vi "AutoInstaller.vi"() -> ()   [LabVIEW 2020]
uses:
  <vilib>/zip/NI_Unzip.lvlib
panel:
  out "Text":string
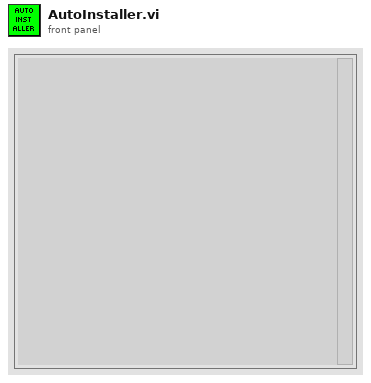
[diagram p1: front panel]
types:
  T1 = cluster{"BuildFolder":path, "Files":cluster{"ZipFile":path, "UnzippedFolder":path, "LVPath":path, "LvVer":i32, "Bit":i32}[], "LogFile":path, "pattern":string}
  T2 = cluster{"ZipFile":path, "UnzippedFolder":path, "LVPath":path, "LvVer":i32, "Bit":i32}
  T3 = cluster{"ZipFile":path, "UnzippedFolder":path, "LVPath":path, "LvVer":i32, "Bit":i32}[]
  T4 = enum32{"invalid app kind", "Development System", "Run Time System", "Student Edition", "Embedded LabVIEW", "Evaluation", "Custom"}
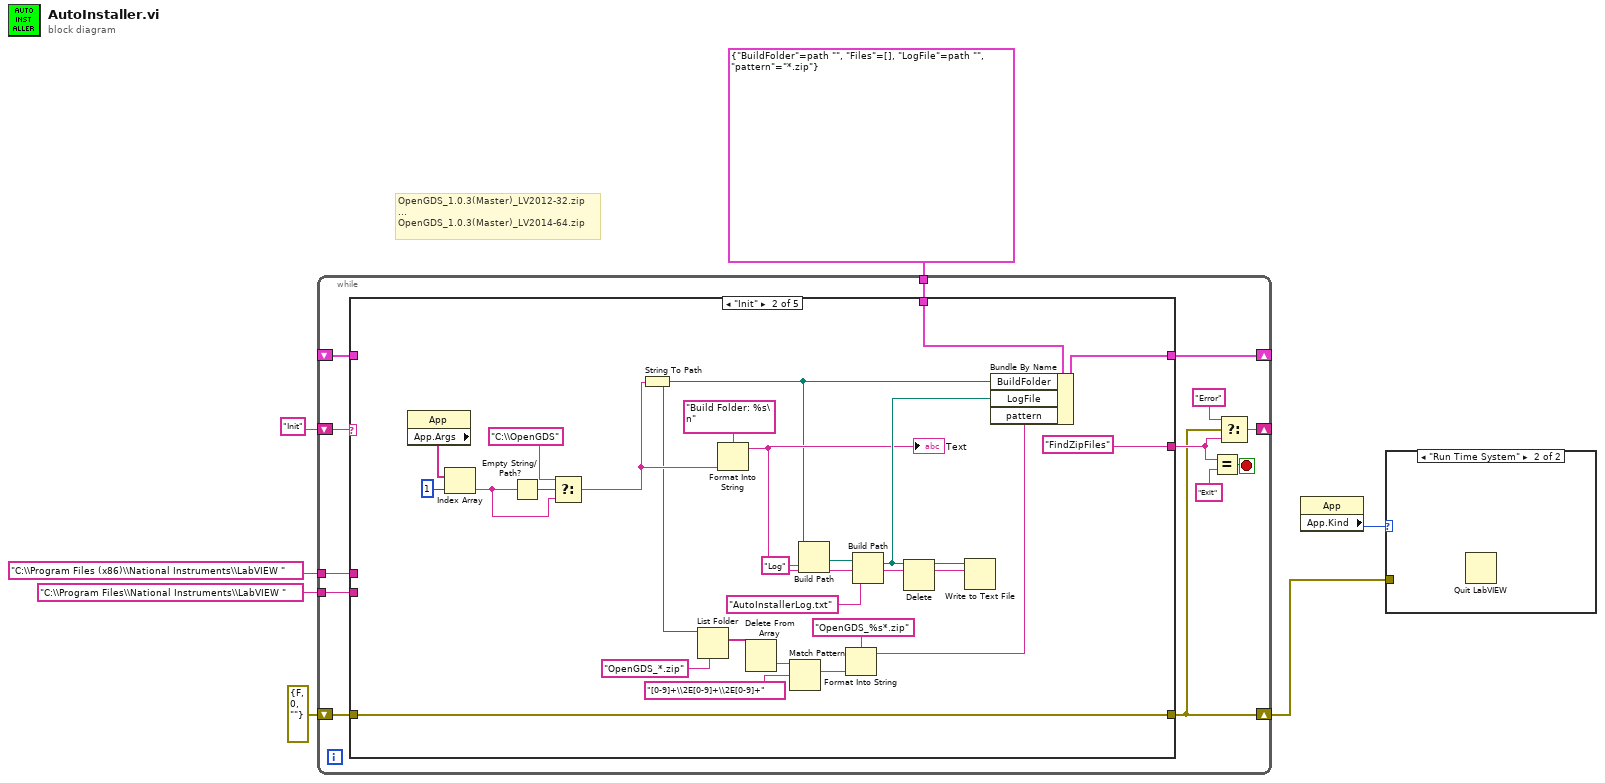
[diagram p0: block diagram]
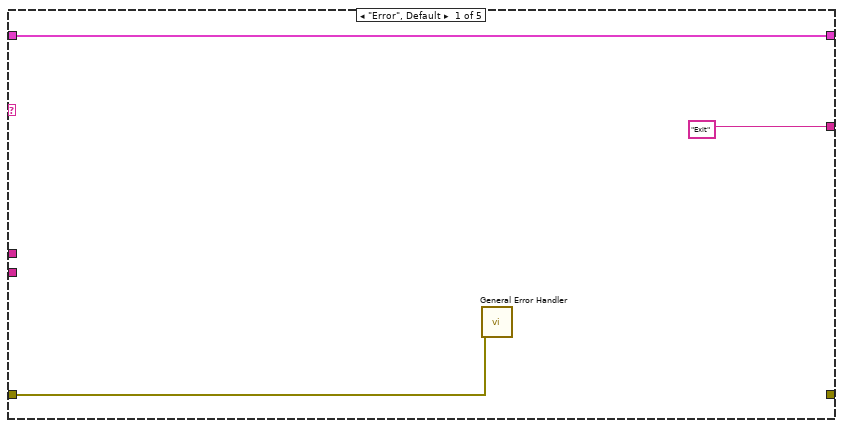
[diagram p3: hidden frame]
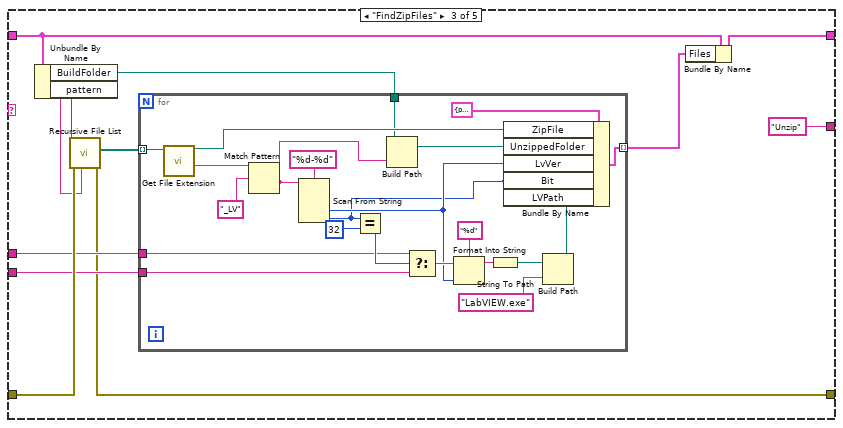
[diagram p4: hidden frame]
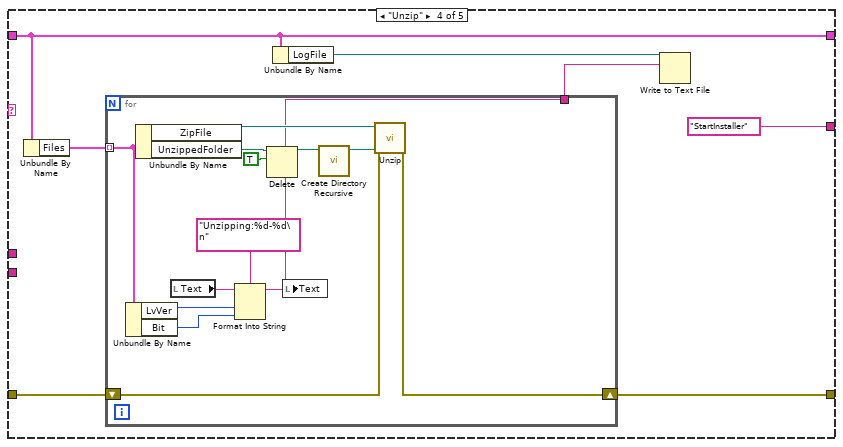
[diagram p5: hidden frame]
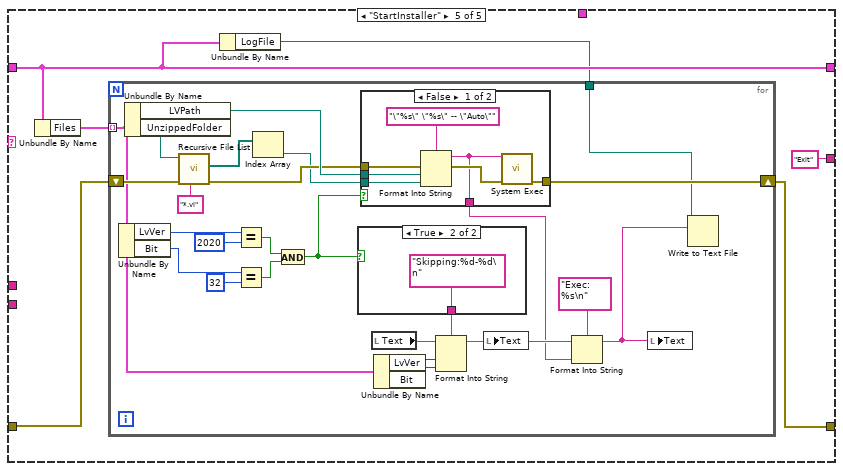
[diagram p6: hidden frame]
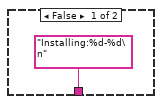
[diagram p7: hidden frame]
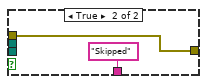
[diagram p8: hidden frame]
diagram:
  # "OpenGDS_1.0.3(Master)_LV2012-32.zip\n...\nOpenGDS_1.0.3(Master)_LV2014-64.zip"
  n1 = while {
    shift-right: [w13] -> w1
    shift-left: errorcluster {"status"=FALSE, "code"=0, "source"=""} ("error IO") -> [w20]
    shift-right: [w18] -> _
    shift-left: "Init" -> [w19]
    shift-right: [w12] -> _
    shift-left: _ -> [w11]
    tunnel: T1 {"BuildFolder"=path "", "Files"=[], "LogFile"=path "", "pattern"="*.zip"} -> [w10]
    tunnel: "C:\\Program Files (x86)\\National Instruments\\LabVIEW " -> [w9]
    tunnel: "C:\\Program Files\\National Instruments\\LabVIEW " -> [w8]
    stop <- w17 stop-if-true
    n2 = case shown="\"Init\"" w19 {
      tunnel: w20 -> [w21 w47 w56 w86 w106]
      tunnel: [_ w47 w51 w85 w104] -> w13
      tunnel: ["Exit" "FindZipFiles" "Unzip" "StartInstaller" "Exit"] -> w14
      tunnel: [w22 w46 w57 w84 w103] -> w12
      tunnel: w11 -> [w22 _ w58 w84 w103]
      tunnel: w10 -> [_ w42 _ _ _]
      tunnel: w9 -> [_ _ w54 _ _]
      tunnel: w8 -> [_ _ w53 _ _]
      frame "Error", Default {
        n3 = call <vilib>:"General Error Handler.vi"("error in (no error)"=w21) -> ()  [unwired: 10 in, 5 out]
      }
      frame "Init" {
        n4 = property class="App"() -> ("App.Args"=w43:string[])  [unwired: 2 in, 2 out]
        n5 = Index Array(array=w43, index=1) -> (element=w40:string)
        n6 = Empty String/Path?(string/path=w40) -> (empty?=w41:bool)
        n7 = Select(t="C:\\OpenGDS", s=w41, f=w40) -> (s? t:f=w39:string)
        n8 = String To Path(string=w39) -> (path=w31:path)
        n9 = List Folder(path=w31, pattern="OpenGDS_*.zip") -> (filenames=w24:string[])  [unwired: 2 in, 3 out]
        n10 = Format Into String(format string="Build Folder: %s\n", w39) -> (resulting string=w32:string)  [unwired: 2 in, 1 out]
        "Text" <- w32
        n11 = Delete From Array(array=w24) -> (deleted portion=w29:string)  [unwired: 2 in, 1 out]
        n12 = Match Pattern(string=w29, regular expression="[0-9]+\\2E[0-9]+\\2E[0-9]+") -> (match substring=w27:string)  [unwired: 1 in, 3 out]
        n13 = Build Path(base path=w31, name or relative path="Log") -> (appended path=w36:path)
        n14 = Format Into String(format string="OpenGDS_%s*.zip" ("name or relative path"), w27) -> (resulting string=w25:string)  [unwired: 2 in, 1 out]
        n15 = Build Path(base path=w36, name or relative path="AutoInstallerLog.txt") -> (appended path=w33:path)
        n16 = Delete(path (use dialog)=w33) -> (deleted path=w34:path)  [unwired: 4 in, 2 out]
        n17 = Write to Text File(file (use dialog)=w34, text=w32) -> ()  [unwired: 2 in, 3 out]
        n18 = Bundle By Name(cluster=w42, "BuildFolder"=w31, "LogFile"=w33, "pattern"=w25) -> (w46:T1)
      }
      frame "FindZipFiles" {
        n19 = Unbundle By Name(w58) -> ("BuildFolder"=w50:path, "pattern"=w49:string)
        n20 = call <vilib>:"Recursive File List.vi"("pattern"=w49, "error in (no error)"=w56, "Folder Path"=w50) -> ("error out"=w51:errorcluster, "All Files in Dir"=w55:path[])  [unwired: 4 in, 3 out]
        n21 = for {
          tunnel: w55 -> [w81] mode=indexing
          tunnel: w54 -> [w76]
          tunnel: w53 -> [w75]
          tunnel: [w65] -> w52 mode=indexing
          tunnel: w50 -> [w64]
          n22 = call <vilib>:"Get File Extension.vi"("file"=w81) -> ("filename without extension"=w60:string, "dup file"=w69:path)  [unwired: 6 in, 3 out]
          n23 = Match Pattern(string=w60, regular expression="_LV") -> (after substring=w68:string)  [unwired: 1 in, 3 out]
          n24 = Scan From String(format string="%d-%d", input string=w68) -> (output 1=w62:i32, output 2=w61:i32)  [unwired: 4 in, 3 out]
          n25 = Equal?(x=w61, y=32) -> (x = y?=w77:bool)
          n26 = Build Path(base path=w64, name or relative path=w68) -> (appended path=w67:path)
          n27 = Select(t=w76, s=w77, f=w75) -> (s? t:f=w74:string)
          n28 = Format Into String(format string="%d", initial string=w74, w62) -> (resulting string=w72:string)  [unwired: 1 in, 1 out]
          n29 = String To Path(string=w72) -> (path=w71:path)
          n30 = Build Path(base path=w71, name or relative path="LabVIEW.exe") -> (appended path=w66:path)
          n31 = Bundle By Name(cluster=T2 {"ZipFile"=path "", "UnzippedFolder"=path "", "LVPath"=path "", "LvVer"=0, "Bit"=0}, "ZipFile"=w69, "UnzippedFolder"=w67, "LvVer"=w62, "Bit"=w61, "LVPath"=w66) -> (w65:T2)
        }
        n32 = Bundle By Name(cluster=w58, "Files"=w52) -> (w57:T1)
      }
      frame "Unzip" {
        n33 = Unbundle By Name(w84) -> ("Files"=w87:T3)
        n34 = for {
          tunnel: w87 -> [w92] mode=indexing
          shift-right: [w99] -> w85
          shift-left: w86 -> [w100]
          tunnel: [w89] -> w82
          n35 = Unbundle By Name(w92) -> ("LvVer"=w91:i32, "Bit"=w90:i32)
          n36 = Unbundle By Name(w92) -> ("ZipFile"=w101:path, "UnzippedFolder"=w98:path)
          n37 = local read "Text"() -> (w94:string)
          n38 = Format Into String(format string="Unzipping:%d-%d\n", initial string=w94, w91, w90) -> (resulting string=w89:string)  [unwired: 1 in, 1 out]
          n39 = Delete(path (use dialog)=w98, entire hierarchy (F)=TRUE) -> (deleted path=w96:path)  [unwired: 3 in, 2 out]
          n40 = local write "Text"(w89) -> ()
          n41 = call <vilib>:"Create Directory Recursive.vi"("directory"=w96) -> ("directory copy"=w95:path)  [unwired: 4 in, 2 out]
          n42 = call <vilib>:"Unzip.vi"("error in (no error)"=w100, "Target directory (same as Zip file if empty)"=w95, "Zip file"=w101) -> ("error out"=w99:errorcluster)  [unwired: 6 in, 2 out]
        }
        n43 = Unbundle By Name(w84) -> ("LogFile"=w83:path)
        n44 = Write to Text File(file (use dialog)=w83, text=w82) -> ()  [unwired: 2 in, 3 out]
      }
      frame "StartInstaller" {
        n45 = Unbundle By Name(w103) -> ("Files"=w107:T3)
        n46 = Unbundle By Name(w103) -> ("LogFile"=w102:path)
        n47 = for {
          tunnel: w107 -> [w118] mode=indexing
          shift-right: [w129] -> w104
          shift-left: w106 -> [w131]
          tunnel: w102 -> [w117]
          n48 = Unbundle By Name(w118) -> ("LvVer"=w124:i32, "Bit"=w121:i32)
          n49 = Unbundle By Name(w118) -> ("LVPath"=w127:path, "UnzippedFolder"=w132:path)
          n50 = call <vilib>:"Recursive File List.vi"("pattern"="*.vi", "error in (no error)"=w131, "Folder Path"=w132) -> ("error out"=w126:errorcluster, "All Files in Dir"=w128:path[])  [unwired: 4 in, 3 out]
          n51 = Equal?(x=w124, y=2020) -> (x = y?=w120:bool)
          n52 = Equal?(x=w121, y=32) -> (x = y?=w119:bool)
          n53 = Index Array(array=w128) -> (element=w125:path)  [unwired: 1 in]
          n54 = And(x=w120, y=w119) -> (x .and. y?=w112:bool)
          n55 = case shown="True" w112 {
            tunnel: ["Installing:%d-%d\n" ("format string") "Skipping:%d-%d\n" ("format string")] -> w115
            frame False {
            }
            frame True {
            }
          }
          n56 = case shown="False" w112 {
            tunnel: [w141 w143] -> w129
            tunnel: w127 -> [w140 _]
            tunnel: w126 -> [w139 w143]
            tunnel: w125 -> [w138 _]
            tunnel: [w135 "Skipped"] -> w108
            frame False {
              n57 = Format Into String(format string="\"%s\" \"%s\" -- \"Auto\"", error in=w139, w140, w138) -> (resulting string=w135:string, error out=w136:errorcluster)  [unwired: 1 in]
              n58 = call <vilib>:"System Exec.vi"("error in (no error)"=w136, "command line"=w135) -> ("error out"=w141:errorcluster)  [unwired: 6 in, 3 out]
            }
            frame True {
            }
          }
          n59 = local read "Text"() -> (w116:string)
          n60 = Unbundle By Name(w118) -> ("LvVer"=w114:i32, "Bit"=w113:i32)
          n61 = Format Into String(format string=w115, initial string=w116, w114, w113) -> (resulting string=w111:string)  [unwired: 1 in, 1 out]
          n62 = local write "Text"(w111) -> ()
          n63 = Format Into String(format string="Exec: %s\n", initial string=w111, w108) -> (resulting string=w110:string)  [unwired: 1 in, 1 out]
          n64 = local write "Text"(w110) -> ()
          n65 = Write to Text File(file (use dialog)=w117, text=w110) -> ()  [unwired: 2 in, 3 out]
        }
      }
    }
    n66 = Equal?(x=w14, y="Exit") -> (x = y?=w17:bool)
    n67 = Select(t="Error", s=w13, f=w14) -> (s? t:f=w18:string)
  }
  n68 = property class="App"() -> ("App.Kind"=w2:T4)  [unwired: 2 in, 2 out]
  n69 = case shown="\"Run Time System\"" w2 {
    tunnel: w1 -> [_ _]
    frame Default {
    }
    frame "Run Time System" {
      n70 = Quit LabVIEW() -> ()  [unwired: 1 in]
    }
  }
